vi "set ACLR Power.vi"(8 "error in (no error)":errorcluster, 10 "ACLR Param":T1={"Bandwidth"=0.0, "Offset"=0.0, "Tx Channel Count"=1} {"Tx Channel Count" min=1; "Offset" format="%#_6p"; "Bandwidth" format="%#_6p"}, 11 "FSV-40N in":refnum<class "FSV-40N.lvclass">) -> (0 "error out":errorcluster, 3 "FSV-40N out":refnum<class "FSV-40N.lvclass">)   [LabVIEW 2023, in "Spectrum Analyzer.lvlib" / "FSV-40N.lvclass"]
uses:
  FSV-40N.lvclass
  TYPE DEFINITION/TYPE ACLR Setting Param.ctl
  FSV-40N.lvclass/FSV-40N.ctl
  Spectrum Analyzer.lvlib
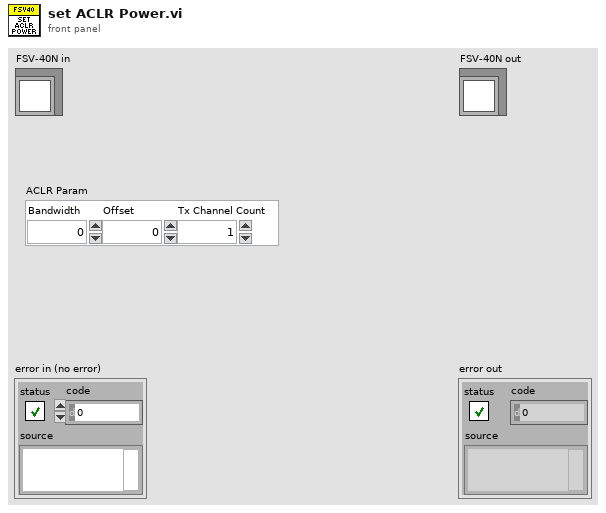
[diagram p1: front panel]
types:
  T1 = typedef "Spectrum Analyzer.lvlib/TYPE ACLR Setting Param.ctl" = cluster{"Bandwidth":dbl, "Offset":dbl, "Tx Channel Count":i32}
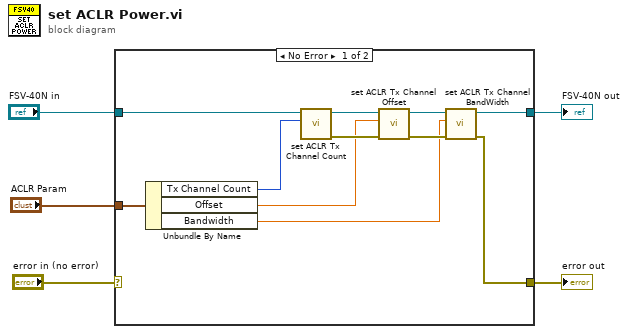
[diagram p0: block diagram]
diagram:
  n1 = case shown="No Error" "error in (no error)" {
    selector: "error in (no error)" -> [_ w17]
    tunnel: "FSV-40N in" -> [w15 w18]
    tunnel: [w8 w18] -> w3
    tunnel: [w6 w17] -> w2
    tunnel: "ACLR Param" -> [w16 _]
    frame No Error {
      n2 = Unbundle By Name(w16) -> ("Tx Channel Count"=w14:i32, "Offset"=w11:dbl, "Bandwidth"=w7:dbl)
      n3 = call "set ACLR Tx Channel Count.vi"("Tx Channel Count"=w14, "FSV-40N in"=w15) -> ("error out"=w12:errorcluster, "FSV-40N out"=w13:refnum<class "FSV-40N.lvclass">)  [unwired: 8 in]
      n4 = call "set ACLR Tx Channel Offset.vi"("error in (no error)"=w12, "Tx Channel Offset (Hz)"=w11, "FSV-40N in"=w13) -> ("error out"=w9:errorcluster, "FSV-40N out"=w10:refnum<class "FSV-40N.lvclass">)  [unwired: 7 in]
      n5 = call "set ACLR Tx Channel BandWidth.vi"("error in (no error)"=w9, "Tx Channel BandWidth (Hz)"=w7, "FSV-40N in"=w10) -> ("error out"=w6:errorcluster, "FSV-40N out"=w8:refnum<class "FSV-40N.lvclass">)  [unwired: 7 in]
    }
    frame Error {
    }
  }
  "error out" <- w2
  "FSV-40N out" <- w3
